vi "Generate Lithography Data.vi"(8 "error in (no error)":errorcluster, 11 "Tool Data in":refnum<class "Tool Data.lvclass">) -> (0 "error out":errorcluster, 2 "Lithography Data":T2(array[cluster]), 3 "Tool Data out":refnum<class "Tool Data.lvclass">)   [LabVIEW 2019, in "Tool Data.lvclass"]
uses:
  Tool Data.lvclass
  <userlib>/LevyLab/Relay Box/Typedefs/Resistor--enum.ctl
  Tool Data.lvclass/Tool Data.ctl
  Settings/ObjectSettings/ObjectSettings.lvclass/ObjectSettings.ctl
  Settings/Dot Settings/Dot Settings.lvclass
  C:/Users/Albro/Documents/GitHub/AFM-Lithography/lvsrc/Classes/Settings/ObjectSettings/ObjectSettings.lvclass
  Settings/Rectangle Settings/Rectangle Settings.lvclass
  Settings/Funnel Settings/Funnel Settings.lvclass
  Settings/Path Settings/Path Settings.lvclass
  Tool Path/Tool Path.lvclass
  Tool Funnel/Tool Funnel.lvclass
  Tool Rectangle/Tool Rectangle.lvclass
  Tool Dot/Tool Dots.lvclass
  Settings/ObjectSettings/ObjectSettings.lvclass
  <userlib>/LevyLab/Relay Box/Relay-Box.lvclass
  Identity/Identifier.lvclass
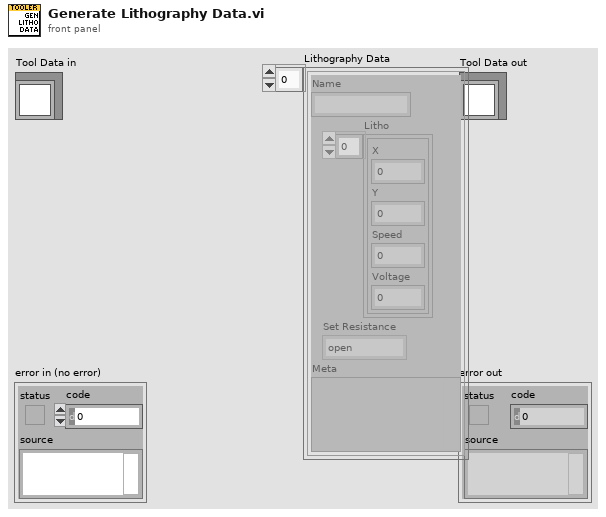
[diagram p1: front panel]
types:
  T1 = typedef "Relay-Box.lvclass/Resistor--enum.ctl" = enum16{"open", "discharge tip", "0 ohms", "100k ohm", "10M ohm", "1G ohm"}
  T2 = cluster{"Name":string, "Litho":cluster{"X":dbl, "Y":dbl, "Speed":dbl, "Voltage":dbl}[], "Set Resistance":T1, "Meta":variant}[]
  T3 = cluster{"Name":string, "Litho":cluster{"X":dbl, "Y":dbl, "Speed":dbl, "Voltage":dbl}[], "Set Resistance":T1, "Meta":variant}
  T4 = cluster{"X":dbl, "Y":dbl, "Speed":dbl, "Voltage":dbl}[]
  T5 = enum16{"Open", "Discharge Tip", "0 ohm", "100 kohm", "10 Mohm", "1 Gohm"}
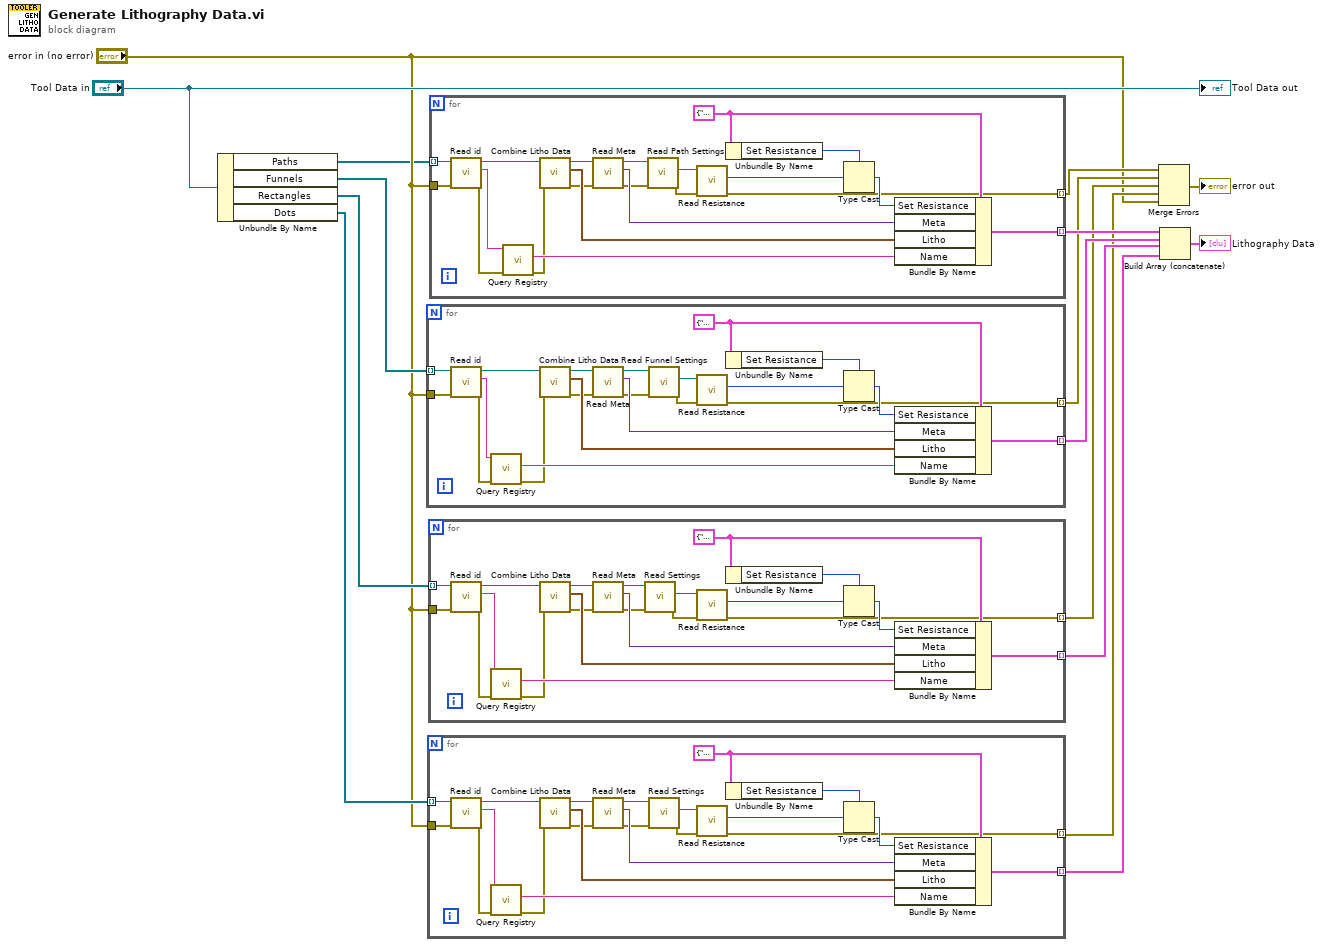
[diagram p0: block diagram]
diagram:
  n1 = Unbundle By Name("Tool Data in") -> ("Paths"=w1:refnum<class "Tool Path.lvclass">[], "Funnels"=w15:refnum<class "Tool Funnel.lvclass">[], "Rectangles"=w14:refnum<class "Tool Rectangle.lvclass">[], "Dots"=w13:refnum<class "Tool Dots.lvclass">[])
  n2 = for {
    tunnel: w15 -> [w23] mode=indexing
    tunnel: [w30] -> w11 mode=indexing
    tunnel: "error in (no error)" -> [w21]
    tunnel: [w27] -> w7 mode=indexing
    w33 = T3 {"Name"="", "Litho"=[], "Set Resistance"=enum."1G ohm", "Meta"=variant} ("Pattern Data")
    n3 = call-dynamic "Read id.vi"("error in (no error)"=w21, "Tool Path in"=w23) -> ("error out"=w17:errorcluster, "id"=w20:string, "Tool Path out"=w22:refnum<class "Tool Funnel.lvclass">)  [unwired: 7 in]
    n4 = call "Query Registry.vi"("error in"=w17, "Name In"=w20) -> ("error out"=w18:errorcluster, "Alias"=w19:string)  [unwired: 6 in, 2 out]
    n5 = call-dynamic "Combine Litho Data.vi"("error in (no error)"=w18, "Tool Object in"=w22) -> ("error out"=w26:errorcluster, "Output"=w36:T4, "Tool Object out"=w37:refnum<class "Tool Funnel.lvclass">)  [unwired: 7 in]
    n6 = call-dynamic "Read Meta.vi"("error in (no error)"=w26, "Tool Object in"=w37) -> ("error out"=w25:errorcluster, "Meta"=w35:variant, "Tool Object out"=w29:refnum<class "Tool Funnel.lvclass">)  [unwired: 7 in]
    n7 = call-dynamic "Read Funnel Settings.vi"("error in (no error)"=w25, "Tool Funnel in"=w29) -> ("error out"=w24:errorcluster, "Funnel Settings.lvclass"=w28:refnum<class "Funnel Settings.lvclass">)  [unwired: 7 in, 1 out]
    n8 = call "Read Resistance.vi"("error in (no error)"=w24, "ObjectSettings in"=w28) -> ("error out"=w27:errorcluster, "Resistance"=w34:T5)  [unwired: 7 in, 1 out]
    n9 = Unbundle By Name(w33) -> ("Set Resistance"=w32:T1)
    n10 = Type Cast(type=w32, x=w34) -> (*(type *) &x=w31:T1)
    n11 = Bundle By Name(cluster=w33, "Set Resistance"=w31, "Meta"=w35, "Litho"=w36, "Name"=w19) -> (w30:T3)
  }
  n12 = for {
    tunnel: w13 -> [w44] mode=indexing
    tunnel: [w51] -> w9 mode=indexing
    tunnel: "error in (no error)" -> [w42]
    tunnel: [w45] -> w5 mode=indexing
    w54 = T3 {"Name"="", "Litho"=[], "Set Resistance"=enum."1G ohm", "Meta"=variant} ("Pattern Data")
    n13 = call-dynamic "Read id.vi"("error in (no error)"=w42, "Tool Object in"=w44) -> ("error out"=w40:errorcluster, "id"=w41:string, "Tool Object out"=w43:refnum<class "Tool Dots.lvclass">)  [unwired: 7 in]
    n14 = call "Query Registry.vi"("error in"=w40, "Name In"=w41) -> ("error out"=w38:errorcluster, "Alias"=w39:string)  [unwired: 6 in, 2 out]
    n15 = call-dynamic "Combine Litho Data.vi"("error in (no error)"=w38, "Tool Object in"=w43) -> ("error out"=w48:errorcluster, "Output"=w57:T4, "Tool Object out"=w58:refnum<class "Tool Dots.lvclass">)  [unwired: 7 in]
    n16 = call-dynamic "Read Meta.vi"("error in (no error)"=w48, "Tool Object in"=w58) -> ("error out"=w47:errorcluster, "Meta"=w56:variant, "Tool Object out"=w50:refnum<class "Tool Dots.lvclass">)  [unwired: 7 in]
    n17 = call-dynamic "Read Settings.vi"("error in (no error)"=w47, "Tool Dots in"=w50) -> ("error out"=w46:errorcluster, "Dot Settings.lvclass"=w49:refnum<class "Dot Settings.lvclass">)  [unwired: 7 in, 1 out]
    n18 = call "Read Resistance.vi"("error in (no error)"=w46, "ObjectSettings in"=w49) -> ("error out"=w45:errorcluster, "Resistance"=w55:T5)  [unwired: 7 in, 1 out]
    n19 = Unbundle By Name(w54) -> ("Set Resistance"=w53:T1)
    n20 = Type Cast(type=w53, x=w55) -> (*(type *) &x=w52:T1)
    n21 = Bundle By Name(cluster=w54, "Set Resistance"=w52, "Meta"=w56, "Litho"=w57, "Name"=w39) -> (w51:T3)
  }
  n22 = for {
    tunnel: w14 -> [w64] mode=indexing
    tunnel: [w72] -> w10 mode=indexing
    tunnel: "error in (no error)" -> [w59]
    tunnel: [w69] -> w6 mode=indexing
    w75 = T3 {"Name"="", "Litho"=[], "Set Resistance"=enum."1G ohm", "Meta"=variant} ("Pattern Data")
    n23 = call-dynamic "Read id.vi"("error in (no error)"=w59, "Tool Object in"=w64) -> ("error out"=w61:errorcluster, "id"=w63:string, "Tool Object out"=w65:refnum<class "Tool Rectangle.lvclass">)  [unwired: 7 in]
    n24 = call "Query Registry.vi"("error in"=w61, "Name In"=w63) -> ("error out"=w60:errorcluster, "Alias"=w62:string)  [unwired: 6 in, 2 out]
    n25 = call-dynamic "Combine Litho Data.vi"("error in (no error)"=w60, "Tool Object in"=w65) -> ("error out"=w68:errorcluster, "Output"=w78:T4, "Tool Object out"=w79:refnum<class "Tool Rectangle.lvclass">)  [unwired: 7 in]
    n26 = call-dynamic "Read Meta.vi"("error in (no error)"=w68, "Tool Object in"=w79) -> ("error out"=w67:errorcluster, "Meta"=w77:variant, "Tool Object out"=w71:refnum<class "Tool Rectangle.lvclass">)  [unwired: 7 in]
    n27 = call-dynamic "Read Settings.vi"("error in (no error)"=w67, "Tool Rectangle in"=w71) -> ("error out"=w66:errorcluster, "Rectangle Settings.lvclass"=w70:refnum<class "Rectangle Settings.lvclass">)  [unwired: 7 in, 1 out]
    n28 = call "Read Resistance.vi"("error in (no error)"=w66, "ObjectSettings in"=w70) -> ("error out"=w69:errorcluster, "Resistance"=w76:T5)  [unwired: 7 in, 1 out]
    n29 = Unbundle By Name(w75) -> ("Set Resistance"=w74:T1)
    n30 = Type Cast(type=w74, x=w76) -> (*(type *) &x=w73:T1)
    n31 = Bundle By Name(cluster=w75, "Set Resistance"=w73, "Meta"=w77, "Litho"=w78, "Name"=w62) -> (w72:T3)
  }
  n32 = for {
    tunnel: w1 -> [w85] mode=indexing
    tunnel: [w91] -> w12 mode=indexing
    tunnel: "error in (no error)" -> [w84]
    tunnel: [w90] -> w4 mode=indexing
    w94 = T3 {"Name"="", "Litho"=[], "Set Resistance"=enum."1G ohm", "Meta"=variant} ("Pattern Data")
    n33 = call-dynamic "Read id.vi"("error in (no error)"=w84, "Tool Path in"=w85) -> ("error out"=w81:errorcluster, "id"=w83:string, "Tool Path out"=w86:refnum<class "Tool Path.lvclass">)  [unwired: 7 in]
    n34 = call "Query Registry.vi"("error in"=w81, "Name In"=w83) -> ("error out"=w80:errorcluster, "Alias"=w82:string)  [unwired: 6 in, 2 out]
    n35 = call-dynamic "Combine Litho Data.vi"("error in (no error)"=w80, "Tool Object in"=w86) -> ("error out"=w89:errorcluster, "Output"=w97:T4, "Tool Object out"=w100:refnum<class "Tool Path.lvclass">)  [unwired: 7 in]
    n36 = call-dynamic "Read Meta.vi"("error in (no error)"=w89, "Tool Object in"=w100) -> ("error out"=w88:errorcluster, "Meta"=w96:variant, "Tool Object out"=w99:refnum<class "Tool Path.lvclass">)  [unwired: 7 in]
    n37 = call-dynamic "Read Path Settings.vi"("error in (no error)"=w88, "Tool Path in"=w99) -> ("error out"=w87:errorcluster, "Path Settings.lvclass"=w98:refnum<class "Path Settings.lvclass">)  [unwired: 7 in, 1 out]
    n38 = call "Read Resistance.vi"("error in (no error)"=w87, "ObjectSettings in"=w98) -> ("error out"=w90:errorcluster, "Resistance"=w95:T5)  [unwired: 7 in, 1 out]
    n39 = Unbundle By Name(w94) -> ("Set Resistance"=w93:T1)
    n40 = Type Cast(type=w93, x=w95) -> (*(type *) &x=w92:T1)
    n41 = Bundle By Name(cluster=w94, "Set Resistance"=w92, "Meta"=w96, "Litho"=w97, "Name"=w82) -> (w91:T3)
  }
  n42 = Merge Errors(w4, w7, w6, w5, "error in (no error)") -> (→"error out":errorcluster)
  n43 = Build Array (concatenate)(w12, w11, w10, w9) -> (→"Lithography Data":T2)
  "Tool Data out" <- "Tool Data in"
